vi "test_Get Slot.vi"(8 "error in (no error)":errorcluster, 11 "TestCase in":refnum<class "Scan Engine Scripting API Custom Device Unit Tests.lvclass">) -> (0 "error out":errorcluster, 3 "TestCase out":refnum<class "Scan Engine Scripting API Custom Device Unit Tests.lvclass">)   [LabVIEW 2020, in "Scan Engine Scripting API Custom Device Unit Tests.lvclass"]
uses:
  Scan Engine Scripting API Custom Device Unit Tests.lvclass
  Scripting/Modules/NI 9475/NI 9475.lvclass
  C:/Users/nitest/Desktop/Git 2020/niveristand-scan-engine-ethercat-custom-device/Custom Device Source/Scripting/Modules/Module/Module.lvclass
  Scan Engine Scripting API Custom Device Unit Tests.lvclass/Scan Engine Scripting API Custom Device Unit Tests.ctl
  186bb218-53c3-41f0-9cfc-94fa19d4683d.vi
  Shared/Utility/Set Error.vi
  <vilib>/Utility/error.llb/Clear Errors.vi
  Scripting/Utility/Convert Slot Configuration to 9212.vi
  Scripting/Utility/Convert Slot Configuration to 9213.vi
  Includes/Modules.lvlibp/SD Module/SD Module.lvclass
  C:/Users/nitest/Desktop/Git 2020/niveristand-scan-engine-ethercat-custom-device/Includes/Modules.lvlibp/RSI Module/RSI Module.lvclass
  Scripting/Modules/NI 9212/NI 9212.lvclass
  Scripting/Modules/NI 9213/NI 9213.lvclass
  Scripting/Modules/NI 9224/NI 9224.lvclass
  Scripting/Modules/NI 9228/NI 9228.lvclass
  Includes/Modules.lvlibp/RSI Module/Read Module Page Property.vi
  Includes/Modules.lvlibp/RSI Module/Read Model.vi
  Scripting/Utility/Convert Module Model to Module Class.vi
  Includes/Modules.lvlibp/SD Module/Read DIO mode.vi
  Includes/Modules.lvlibp/RSI Module/Read Channels.vi
  Scripting/Utility/Convert to DI Module.vi
  Scripting/Utility/Convert to DO Module.vi
  Scripting/Utility/Convert to CI PWM Module.vi
  Scripting/Utility/Convert to CDO Module.vi
  Scripting/Utility/Convert to PWM Module.vi
  Shared/Globals/Error Strings.vi
  Scripting/Utility/Get Channel Names and Default Values for Slot.vi
  Scripting/Modules/NI 9212/Create NI 9212.vi
  Scripting/Modules/NI 9213/Create NI 9213.vi
  Scripting/Utility/Convert to AI Module.vi
  Scripting/Utility/Convert to AI Vrms Module.vi
  Scripting/Utility/Convert to AI Arms Module.vi
  Scripting/Utility/Convert to DIO Module.vi
  Scripting/Modules/Module/Module.lvclass
  Includes/Modules.lvlibp/9212/9212.lvclass
  Includes/Modules.lvlibp/9213/9213.lvclass
  Includes/Modules.lvlibp/9224/9224.lvclass
  <vilib>/addons/_JKI Toolkits/VI Tester/TestCase.llb/TestCase.lvclass
  Scripting/Scan Engine Scripting.lvlib
  Modules/Module Test Classes/Module Test.lvclass
  C:/Program Files (x86)/National Instruments/LabVIEW 2020/vi.lib/addons/_JKI Toolkits/VI Tester/TestCase.llb/TestCase.lvclass
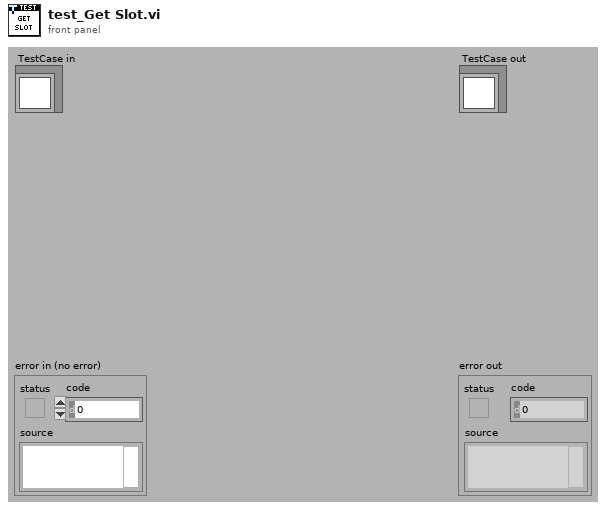
[diagram p1: front panel]
types:
  T1 = typedef "Custom Device API.lvlib/Custom Device Item Ref.ctl" = u64
  T2 = typedef "Scan Engine Scripting.lvlib/Counter Driven Output Mode.lvclass/Drive from Slot.ctl" = enum16{"Slot 1", "Slot 2", "Slot 3", "Slot 4", "Slot 5", "Slot 6", "Slot 7", "Slot 8"}
  T3 = typedef "Scan Engine Scripting.lvlib/counter driven output channel settings.ctl" = cluster{"name":string, "default value":bool, "counter driven state":T4}
  T4 = typedef "Scan Engine Scripting.lvlib/Counter Driven Output Channel.lvclass/Counter Driven State.ctl" = enum16{"Disabled", "Enabled"}
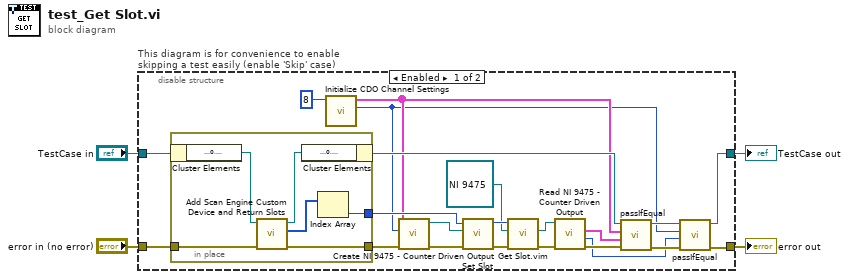
[diagram p0: block diagram]
diagram:
  n1 = disable-structure "This diagram is for convenience to enable skipping a test easily (enable 'Skip' case)" shown="Enabled" {
    disable-tunnel: "TestCase in" -> [w13 w36]
    disable-tunnel: [w20 w34] -> w1
    disable-tunnel: [w11 w35] -> w3
    disable-tunnel: "error in (no error)" -> [w15 w33]
    frame Enabled {
      n2 = in-place {
        in-place-border: [w32] -> w14
        in-place-border: w15 -> [w31]
        in-place-border: [w27] -> w12
        n3 = in-place-cluster #1(w13) -> ("target ref"=w30:refnum<k24>)
        n4 = call "Add Scan Engine Custom Device and Return Slots.vi"("error in"=w31, "target ref in"=w30) -> ("error out"=w32:errorcluster, "slot refs"=w28:T1[], "target ref out"=w29:refnum<k24>)  [unwired: 7 in]
        n5 = in-place-cluster #1("target ref"=w29) -> (w10:refnum<class "Scan Engine Scripting API Custom Device Unit Tests.lvclass">)
        n6 = Index Array(array=w28) -> (element=w27:T1)  [unwired: 1 in]
      }
      n7 = call "Initialize CDO Channel Settings.vi"("array size"=8) -> ("drive from slot"=w5:T2, "channel settings"=w6:T3[])  [unwired: 9 in]
      n8 = call "Create NI 9475 - Counter Driven Output.vi"("error in"=w14, "drive from slot"=w5, "channel settings"=w6) -> ("error out"=w26:errorcluster, "NI 9475 out"=w19:refnum<class "NI 9475.lvclass">)  [unwired: 7 in]
      n9 = call "Set Slot.vi"("error in"=w26, "module"=w19, "slot ref in"=w12) -> ("error out"=w16:errorcluster, "slot ref out"=w24:T1)  [unwired: 7 in]
      n10 = call "Get Slot.vim"("error in"=w16, "module type"=refnum<class "NI 9475.lvclass"> refnum ("NI 9475 out"), "slot ref in"=w24) -> ("error out"=w17:errorcluster, "module"=w18:refnum<class "NI 9475.lvclass">)  [unwired: 5 in, 2 out]
      n11 = call "Read NI 9475 - Counter Driven Output.vi"("error in"=w17, "NI 9475 in"=w18) -> ("error out"=w23:errorcluster, "drive from slot"=w8:T2, "channel settings"=w7:T3[])  [unwired: 6 in, 1 out]
      n12 = call-dynamic "passIfEqual.vi"("error in (no error)"=w23, "y"=w7, "x"=w6, "TestCase in"=w10) -> ("error out"=w22:errorcluster, "TestCase out"=w21:refnum<class "Scan Engine Scripting API Custom Device Unit Tests.lvclass">)  [unwired: 6 in]
      n13 = call-dynamic "passIfEqual.vi"("error in (no error)"=w22, "y"=w8, "x"=w5, "TestCase in"=w21) -> ("error out"=w11:errorcluster, "TestCase out"=w20:refnum<class "Scan Engine Scripting API Custom Device Unit Tests.lvclass">)  [unwired: 6 in]
    }
    frame Disabled {
      # "skip test result while test is under development"
      n14 = call <vilib>:"skip.vi"("error in (no error)"=w33, "TestCase in"=w36) -> ("error out"=w35:errorcluster, "TestCase out"=w34:refnum<class "Scan Engine Scripting API Custom Device Unit Tests.lvclass">)  [unwired: 8 in]
    }
  }
  "error out" <- w3
  "TestCase out" <- w1
